vi "Build VIH Deploy - Progress Indication.vi"(6 "mode (run)":enum16{"run", "start", "stop"}(ring), 8 "error in":errorcluster, 10 "message 2":string, 11 "message 1":string) -> (0 "error out":errorcluster)   [LabVIEW 2014]
doc: "::: VI Helpeks :::\nCopyright (c) 2000-2026 Konstantin Shifershteyn. All rights reserved."
uses:
  <vilib>/Utility/error.llb/Error Cluster From Error Code.vi
  <vilib>/ErrorRing/Error Ring.xnode
panel:
  in  "%Cancel":bool
  out "String":string
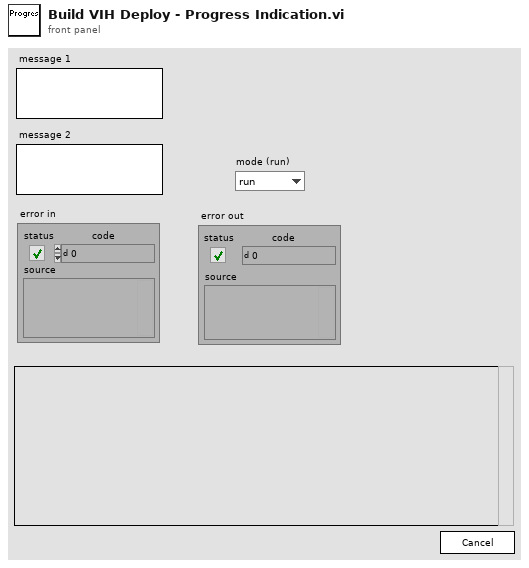
[diagram p1: front panel]
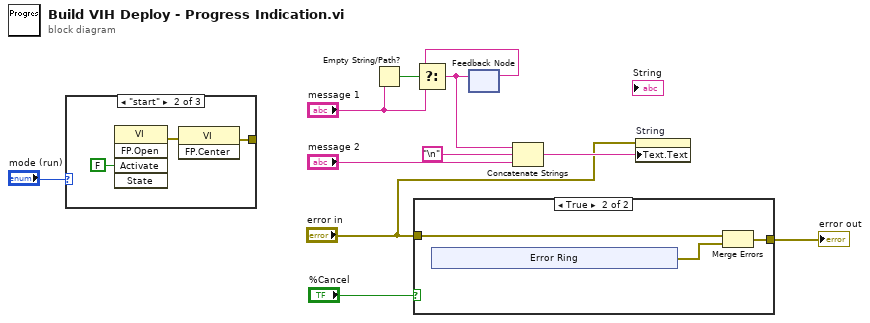
[diagram p0: block diagram]
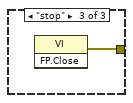
[diagram p4: hidden frame]
diagram:
  n1 = case shown="\"start\"" "mode (run)" {
    tunnel: [_ w12 w15] -> _
    frame "run" {
    }
    frame "start" {
      n2 = invoke class="VI" method="FP.Open"("Activate"=FALSE ("Activate?")) -> (error out=w13:errorcluster)  [unwired: 4 in, 4 out]
      n3 = invoke class="VI" method="FP.Center"(error in=w13) -> (error out=w12:errorcluster)  [unwired: 2 in, 2 out]
    }
    frame "stop" {
      n4 = invoke class="VI" method="FP.Close"() -> (error out=w15:errorcluster)  [unwired: 3 in, 2 out]
    }
  }
  n5 = Empty String/Path?(string/path="message 1") -> (empty?=w10:bool)
  n6 = case shown="True" "%Cancel" {
    tunnel: "error in" -> [w16 w19]
    tunnel: [w16 w18] -> w3
    frame False {
    }
    frame True {
      n7 = xnode "Error Ring"() -> ("error out"=w17:errorcluster)
      n8 = Merge Errors(w19, w17) -> (w18:errorcluster)
    }
  }
  "error out" <- w3
  n9 = feedback #1() -> (w9:string)  [unwired: 1 in]
  n10 = Select(t=w9, s=w10, f="message 1") -> (s? t:f=w8:string)
  n11 = feedback-in #1(w8) -> ()
  n12 = Concatenate Strings(w8, "\n", "message 2") -> (w5:string)
  n13 = property on="String" class="Str"(error in="error in", "Text.Text"=w5) -> ()  [unwired: 1 in, 2 out]
